vi "Set Control Translation.vi"(7 "Obj.":T2={"Type"=enum."Caption", "Translation ANSI"=[], "Translation Unicode"=[]}, 8 "error in (no error)":errorcluster, 9 "Default Lang":i32, 10 "Language":T1, 11 "Control in":refnum<vi>) -> (0 "error out":errorcluster, 3 "Unicode?":bool)   [LabVIEW 2019, in "Language Selection.lvlib"]
doc: "- - -\nCopyright (c) 2026, Merecs Engineering GmbH"
uses:
  Language Selection.lvlib
  TypeDefs/Cluster PropertyTranslation.ctl
  TypeDefs/Enum Property Type.ctl
  TypeDefs/Enum Language.ctl
  <vilib>/Utility/error.llb/Trim Whitespace.vi
  DVR Get Languages.vi
  <vilib>/addons/Tools/Unicode/_subVIs/Convert ASCII to UTF-16LE (1D).vi
  <vilib>/addons/Tools/Unicode/UI Unicode Tools.lvlib
  packages/error-generation/src/Error Generation/Error Generation.lvlib
panel:
  # "Connector Pane"
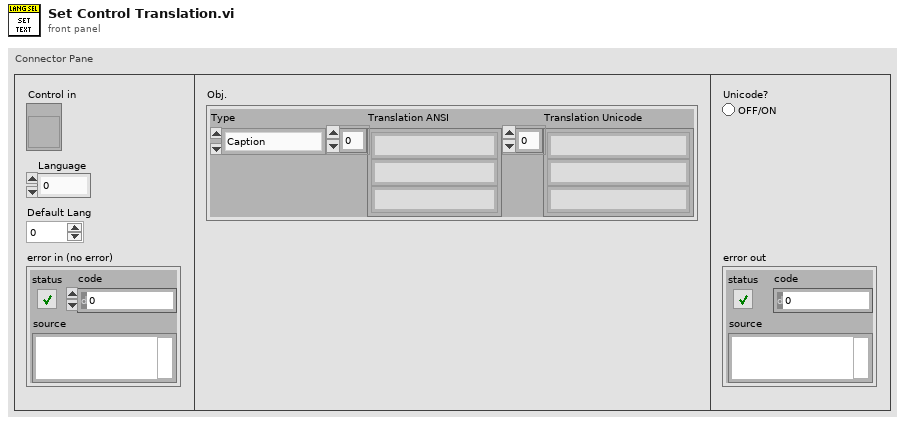
[diagram p1: front panel]
types:
  T1 = typedef "Language Selection.lvlib/Enum Language.ctl" = i32
  T2 = typedef "Language Selection.lvlib/Cluster PropertyTranslation.ctl" = cluster{"Type":T3, "Translation ANSI":string[], "Translation Unicode":string[]}
  T3 = typedef "Language Selection.lvlib/Enum Property Type.ctl" = enum16{"NA", "Caption", "String Value", "Boolean Text", "Ring Strings", "1D Array Elements", "2D Array Elements", "(MC)Listbox Header", "(MC)Listbox Items", "Tab Pages Names", "X & Y GraphChart", "Plot Names", "Table Headers", "Table Items", "TipStrip", "Combobox Strings", "Cursor Name", "Tree Col Headers"}
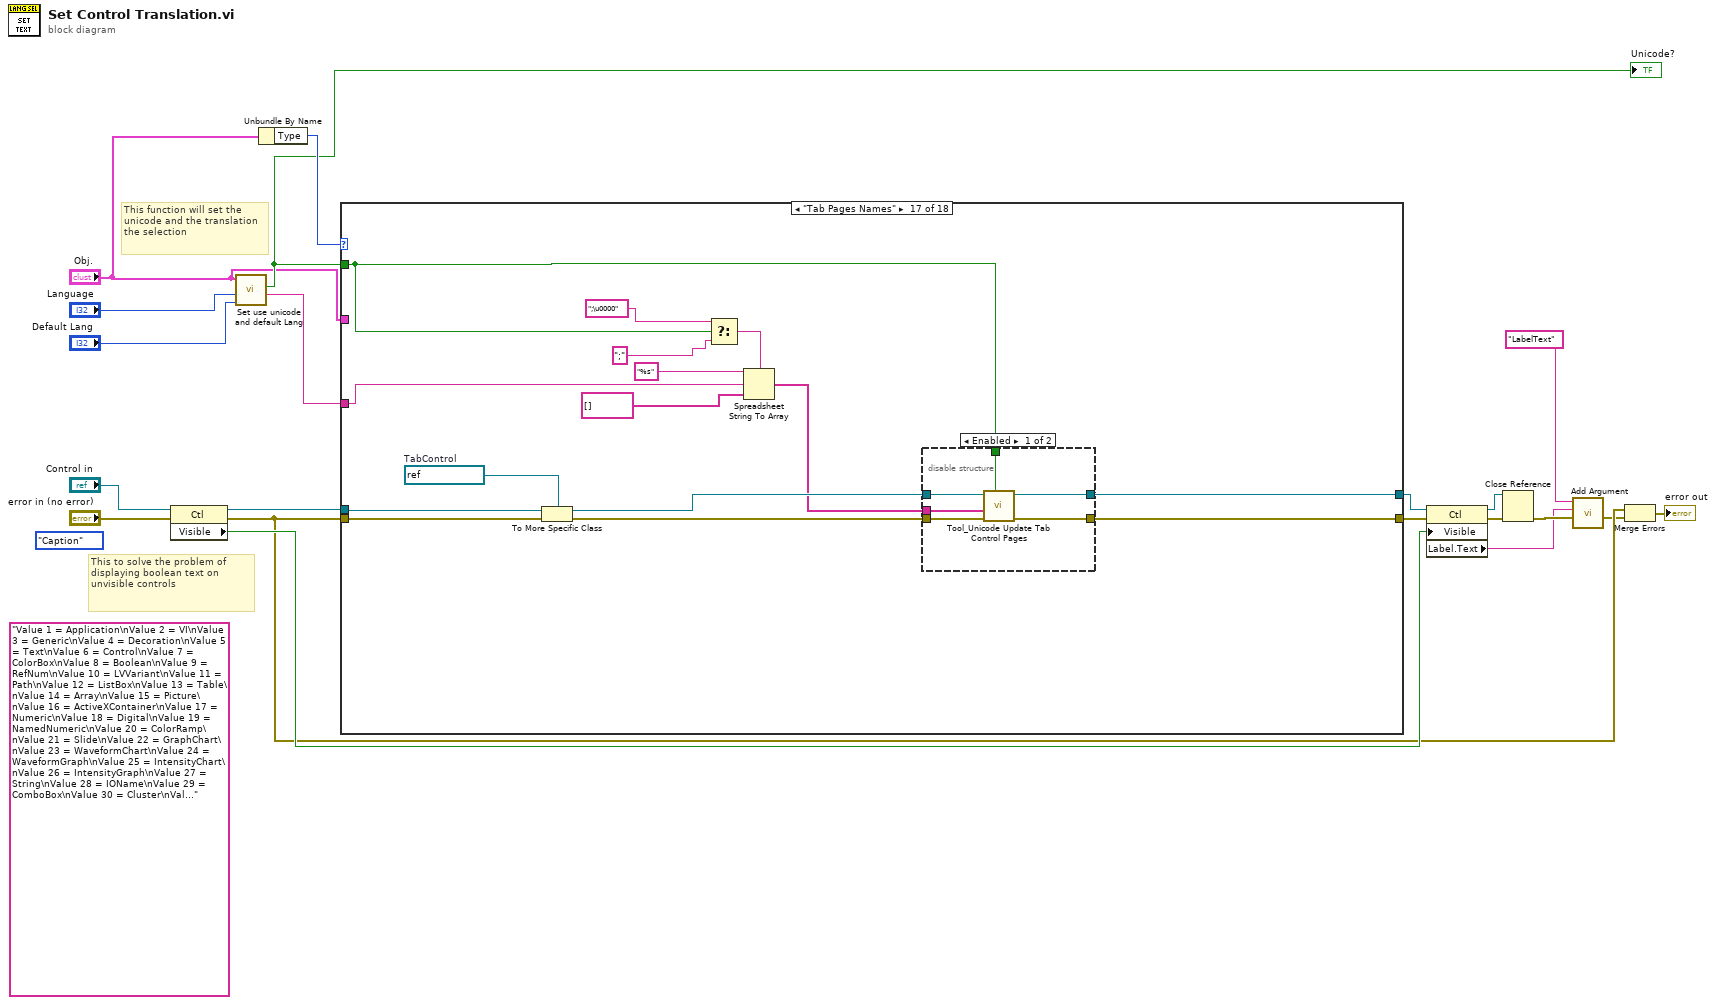
[diagram p0: block diagram]
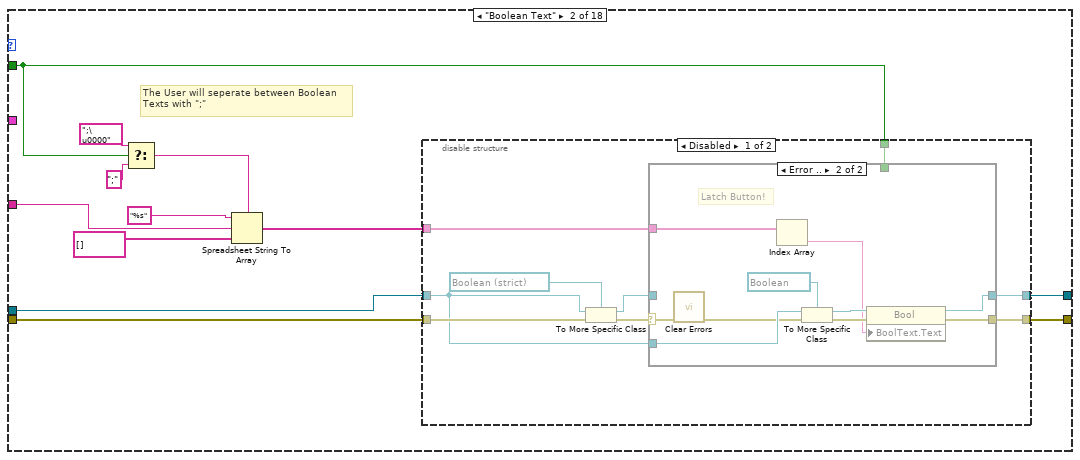
[diagram p3: hidden frame]
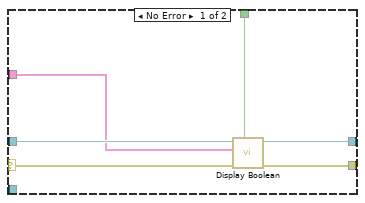
[diagram p4: hidden frame]
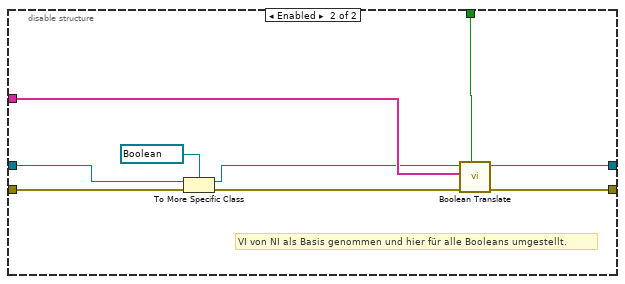
[diagram p5: hidden frame]
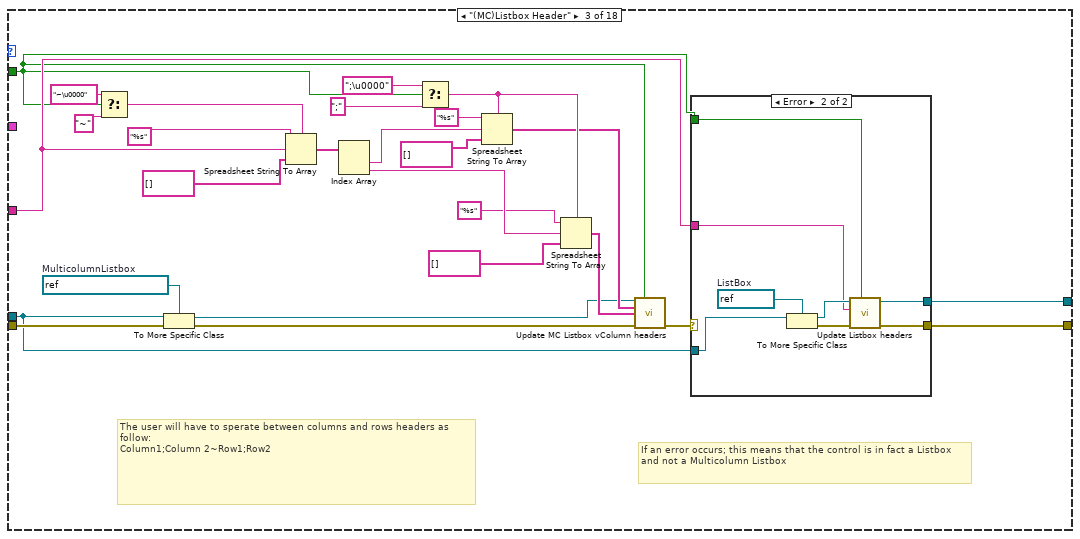
[diagram p6: hidden frame]
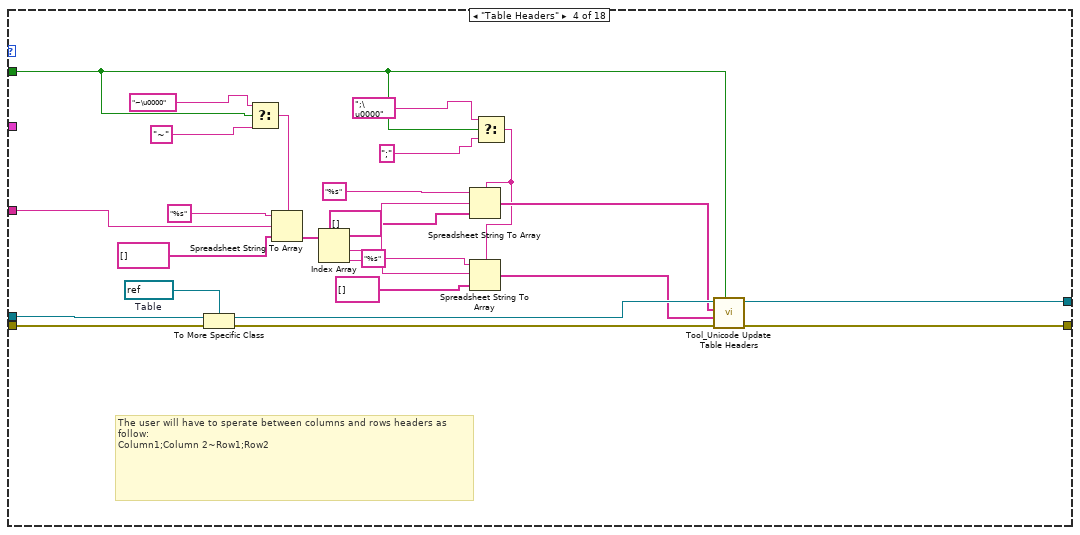
[diagram p8: hidden frame]
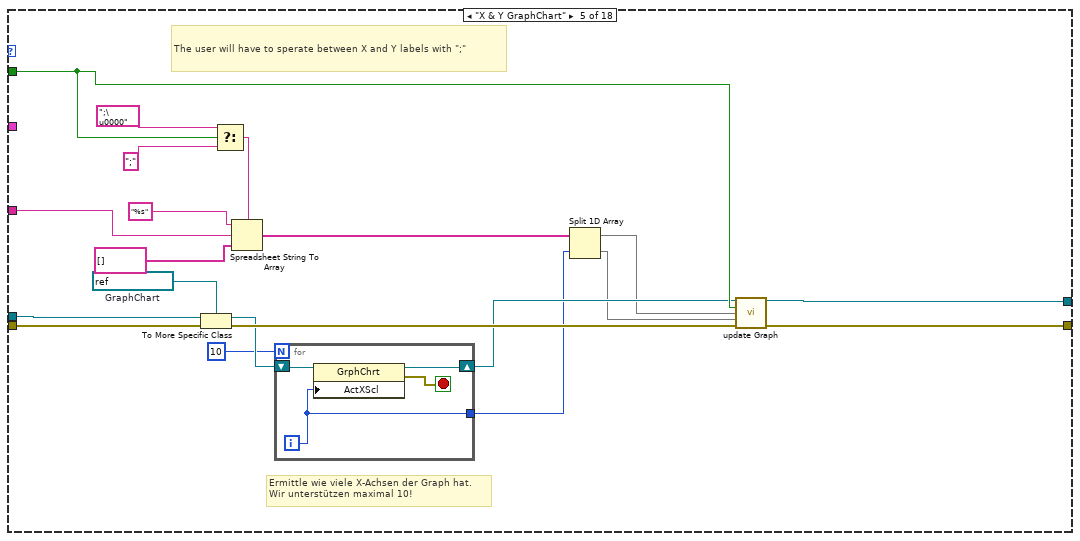
[diagram p9: hidden frame]
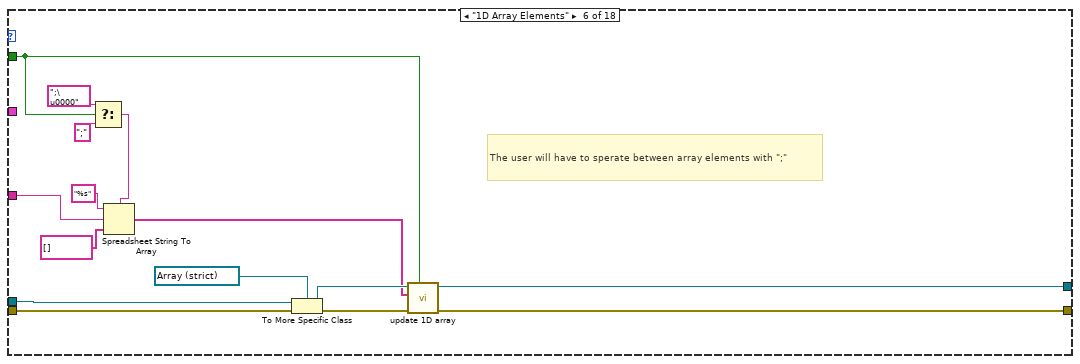
[diagram p10: hidden frame]
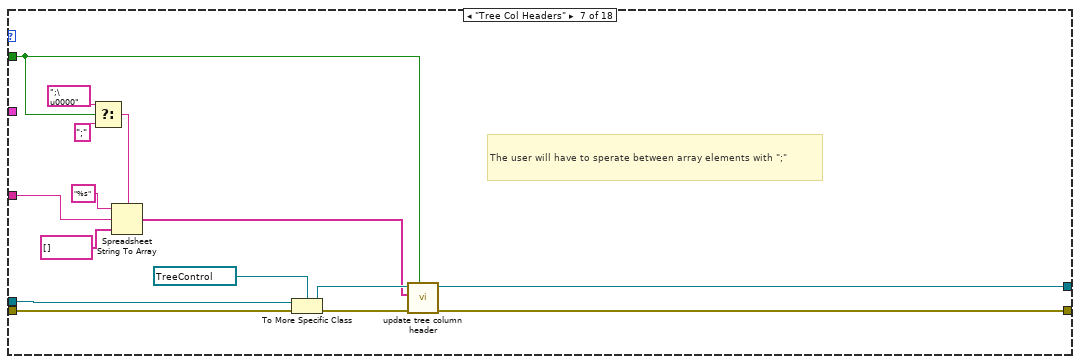
[diagram p11: hidden frame]
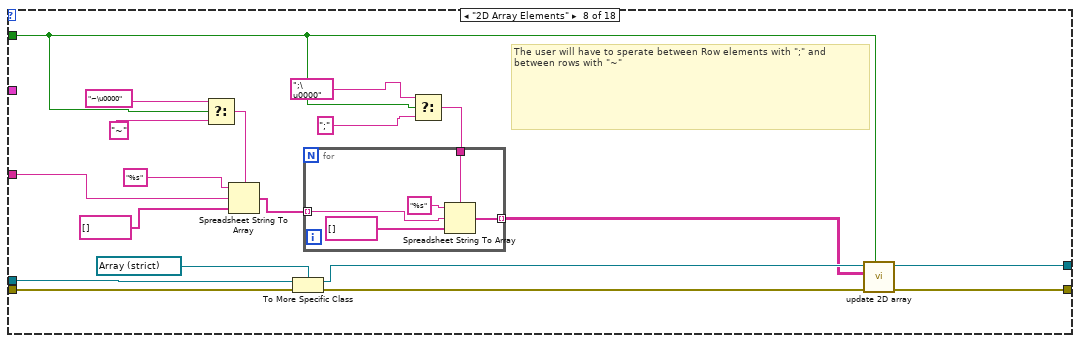
[diagram p12: hidden frame]
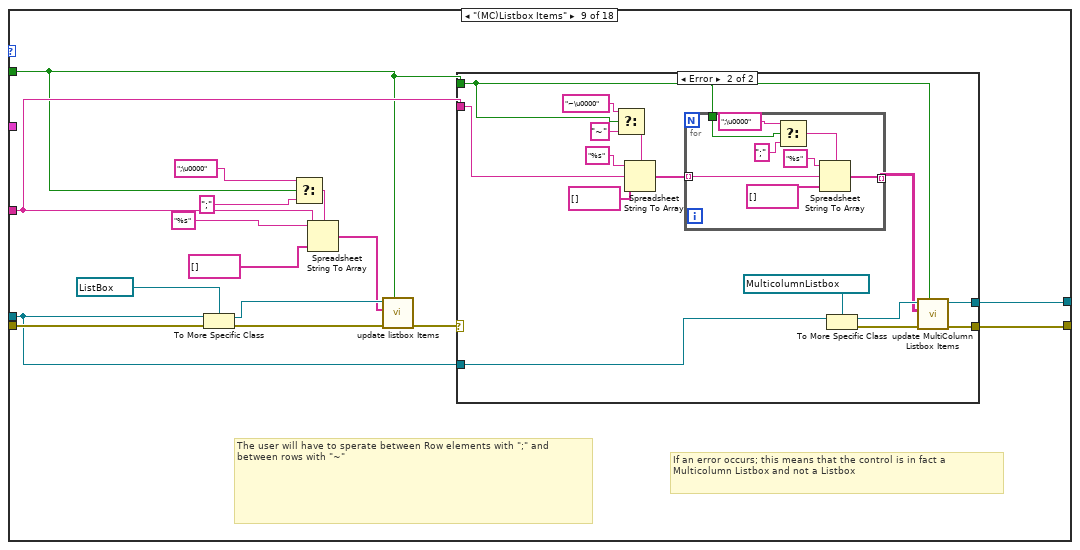
[diagram p13: hidden frame]
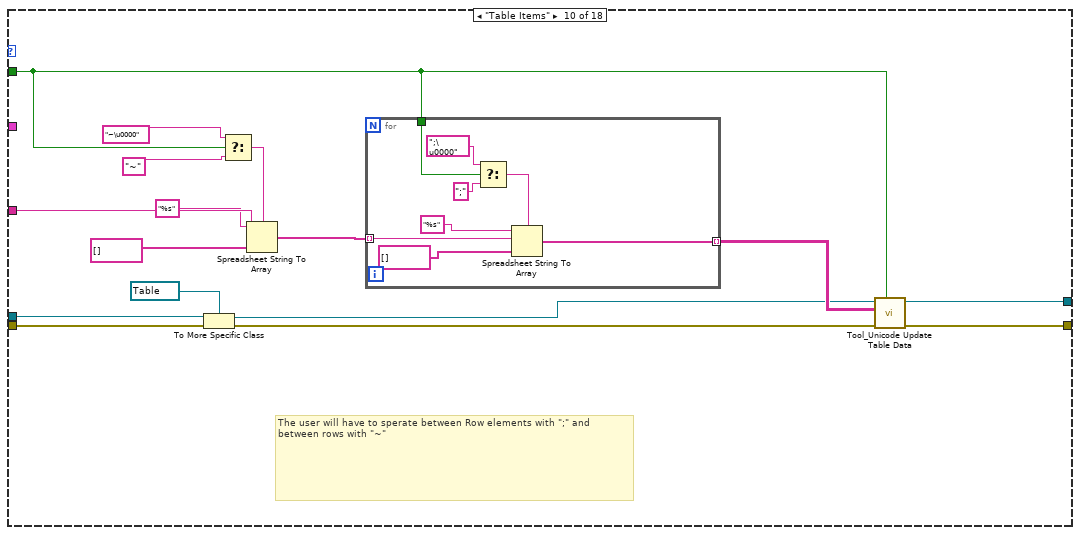
[diagram p15: hidden frame]
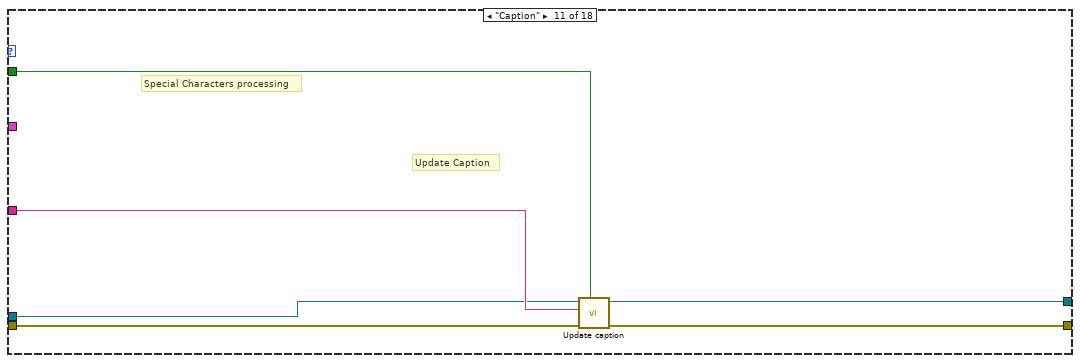
[diagram p16: hidden frame]
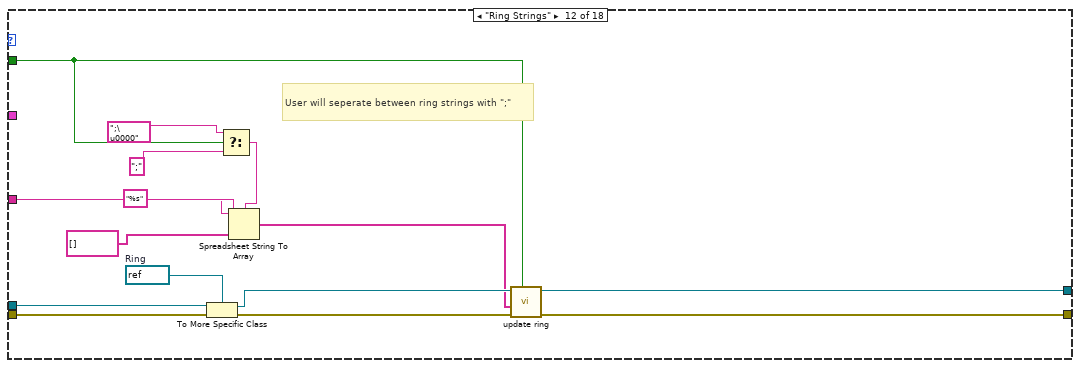
[diagram p17: hidden frame]
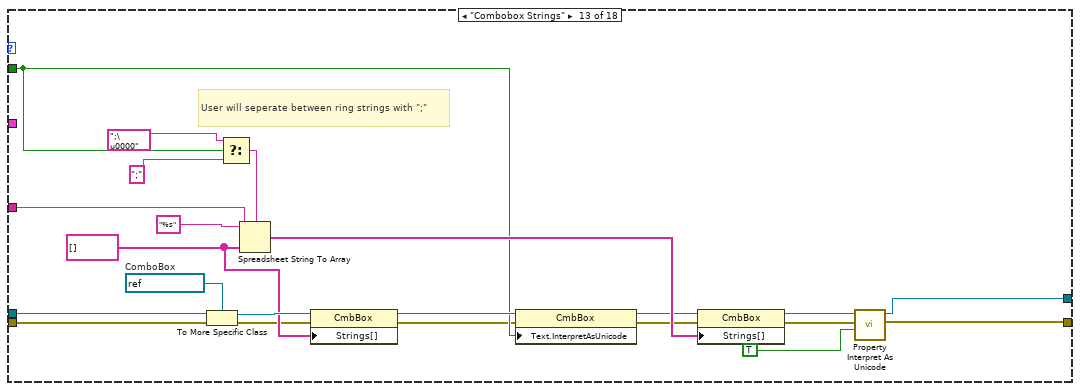
[diagram p18: hidden frame]
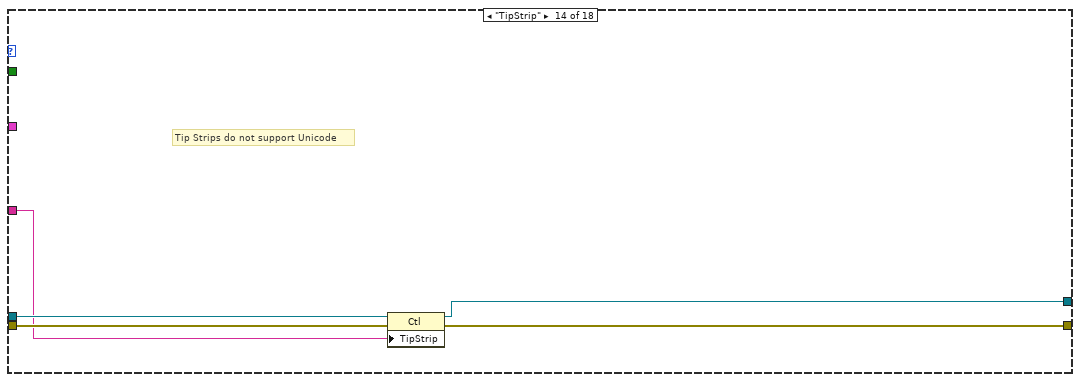
[diagram p19: hidden frame]
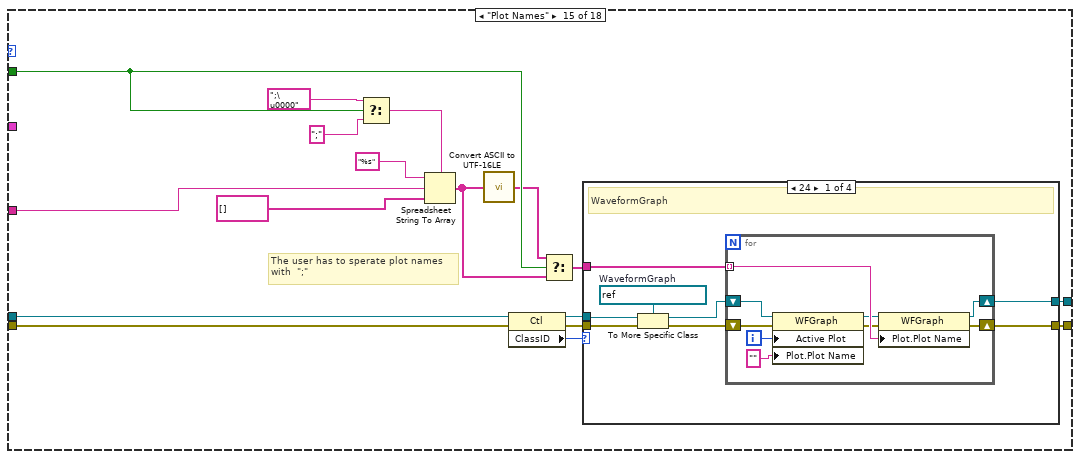
[diagram p20: hidden frame]
diagram:
  (unwired) "Value 1 = Application\nValue 2 = VI\nValue 3 = Generic\nValue 4 = Decoration\nValue 5 = Text\nValue 6 = Control\nValue 7 = ColorBox\nValue 8 = Boolean\nValue 9 = RefNum\nValue 10 = LVVariant\nValue 11 = Path\nValue 12 = ListBox\nValue 13 = Table\nValue 14 = Array\nValue 15 = Picture\nValue 16 = ActiveXContainer\nValue 17 = Numeric\nValue 18 = Digital\nValue 19 = NamedNumeric\nValue 20 = ColorRamp\nValue 21 = Slide\nValue 22 = GraphChart\nValue 23 = WaveformChart\nValue 24 = WaveformGraph\nValue 25 = IntensityChart\nValue 26 = IntensityGraph\nValue 27 = String\nValue 28 = IOName\nValue 29 = ComboBox\nValue 30 = Cluster\nValue 31 = Panel\nValue 32 = Knob\nValue 33 = NumericWithScale\nValue 34 = Ring\nValue 35 = Enum\nValue 36 = GObject\nValue 37 = Plot\nValue 38 = Cursor\nValue 39 = NumericText\nValue 40 = Scale\nValue 41 = ColorScale\nValue 42 = GraphScale\nValue 43 = ColorGraphScale\nValue 44 = TypedRefNum\nValue 45 = Generic\nValue 46 = MulticolumnListbox\nValue 47 = WaveformData\nValue 48 = DSCTag\nValue 49 = DAQChannelName\nValue 50 = VISAResourceName\nValue 51 = IVILogicalName\nValue 52 = SlideScale\nValue 53 = PageSelector\nValue 54 = Page\nValue 55 = TabControl\nValue 56 = ConnectorPane\nValue 57 = DAQmxName\nValue 58 = VIRefNum\nValue 59 = LVObjectRefNum\nValue 60 = AbsTime\nValue 61 = DigitalTable\nValue 62 = SubsystemVI\nValue 63 = Generic\nValue 64 = Generic\nValue 65 = SubPanel\nValue 66 = TreeControl\nValue 67 = GenClassTagRef\nValue 68 = GenClassRef\nValue 69 = RotaryColorScale\nValue 70 = PlugInControl\nValue 71 = PlugInDDODummyContainer\nValue 72 = RadioButtonsControl\nValue 73 = Project\nValue 74 = ProjectItem\nValue 75 = Pane\nValue 76 = Splitter\nValue 77 = BuildSpecification\nValue 78 = Pixmap\nValue 79 = FacadeVI\nValue 80 = Library\nValue 81 = Variable\nValue 82 = TagSet\nValue 83 = XYGraph\nValue 84 = SceneWindow\nValue 85 = LVClassLibrary\nValue 86 = Generic\nValue 87 = MethodVI\nValue 88 = XControlLibrary\nValue 89 = XNodeLibrary\nValue 90 = Scrollbar\nValue 91 = LVTarget\nValue 92 = MixedSignalGraph\nValue 93 = Provider\nValue 94 = CopyOperation\nValue 95 = TargetItem\nValue 96 = ProjectItemType\nValue 97 = CopyItem\nValue 98 = CopyConflict\nValue 99 = CopyExpert\nValue 100 = SceneGraphDisplay\nValue 101 = PolymorphicVI\nValue 102 = LabVIEWClassControl\nValue 103 = XInterfaceLibrary\nValue 104 = SceneNode\nValue 105 = SceneObject\nValue 106 = SceneLight\nValue 107 = Generic\nValue 108 = Generic\nValue 109 = Generic\nValue 110 = SceneClipPlane\nValue 111 = SceneTexture\nValue 112 = SceneGeometry\nValue 113 = SceneBox\nValue 114 = SceneCone\nValue 115 = SceneCylinder\nValue 116 = SceneHeightField\nValue 117 = SceneSphere\nValue 118 = SceneMesh\nValue 119 = XPropertyFolder\nValue 120 = PropertyFolder\nValue 121 = DigitalGraph\nValue 122 = GenClassTagFlatRef\nValue 123 = Scene\nValue 124 = Generic\nValue 125 = LibraryData\nValue 126 = StatechartLibrary\nValue 127 = MixedCheckbox\nValue 128 = SceneDrawable\nValue 129 = SceneText\nValue 130 = MultiSegmentPipe\nValue 131 = Bus\nValue 132 = StubDDO\nValue 133 = ProjectFilesViewItem\nValue 134 = LVClassPropDefFolder\nValue 135 = DataValRefNum"
  (unwired) Enum_Property_Type."Caption" ("Type")
  # "This to solve the problem of displaying boolean text on unvisible controls"
  # "This function will set the unicode and the translation the selection"
  n1 = property class="Ctl"(reference="Control in", error in="error in (no error)") -> (reference out=w13:refnum<vi>, error out=w7:errorcluster, "Visible"=w15:bool)
  n2 = call "Set use unicode and default Lang.vi"("Default Language"="Default Lang", "Startup Language"="Language", "Obj."="Obj.") -> ("Translation out"=w12:string, "Unicode?"=w11:bool)  [unwired: 7 in]
  "Unicode?" <- w11
  n3 = Unbundle By Name("Obj.") -> ("Type"=w20:T3)
  n4 = case shown="\"Tab Pages Names\"" w20 {
    tunnel: w12 -> [_ w33 w89 w127 w145 w168 w183 w203 w217 w265 w277 w288 w313 w318 w323 w411 w423 w447]
    tunnel: w13 -> [w21 w23 w79 w126 w150 w166 w181 w200 w218 w266 w275 w291 w315 w320 w336 w414 w429 w457]
    tunnel: w7 -> [w22 w24 w88 w125 w149 w165 w180 w199 w220 w258 w276 w293 w316 w319 w333 w416 w431 w458]
    tunnel: [w21 w26 w91 w121 w143 w162 w177 w195 w216 w257 w280 w295 w296 w322 w324 w409 w421 w453] -> w18
    tunnel: [w22 w25 w90 w128 w142 w161 w176 w194 w215 w255 w279 w294 w297 w321 w331 w408 w420 w454] -> w19
    tunnel: w11 -> [_ w27 w73 w107 w138 w156 w171 w186 w210 w251 w278 w282 w305 _ w339 w410 w417 w445]
    tunnel: "Obj." -> [_ _ _ _ _ _ _ _ _ _ _ _ _ _ _ _ _ _]
    frame "NA" {
    }
    frame "Boolean Text" {
      # "The User will seperate between Boolean\nTexts with \";\""
      n5 = Select(t=";\u0000" ("delimiter (Tab)"), s=w27, f=";" ("delimiter (Tab)")) -> (s? t:f=w31:string)
      n6 = Spreadsheet String To Array(delimiter (Tab)=w31, format string="%s", spreadsheet string=w33, array type (2D Dbl)=string[] [] ("Strings []")) -> (array=w28:string[])
      n7 = disable-structure shown="Disabled" {
        disable-tunnel: w23 -> [w35 w62]
        disable-tunnel: w28 -> [w43 w68]
        disable-tunnel: w27 -> [w42 w67]
        disable-tunnel: [w41 w66] -> w26
        disable-tunnel: [w40 w65] -> w25
        disable-tunnel: w24 -> [w39 w61]
        frame Disabled {
          n8 = To More Specific Class(target class=refnum<vi> refnum ("Boolean Reference"), reference=w35, error in=w39) -> (specific class reference=w36:refnum<vi>, error out=w38:errorcluster)
          n9 = case shown="Error .." w38 {
            selector: w38 -> [w44 w53]
            tunnel: w36 -> [w49 _]
            tunnel: w43 -> [w48 w51]
            tunnel: w42 -> [w47 _]
            tunnel: [w46 w54] -> w41
            tunnel: [w45 w55] -> w40
            tunnel: w35 -> [_ w56]
            frame No Error {
              n10 = call <vilib>:"Display Boolean.vi"("Interpret as Unicode (T)"=w47, "error in"=w44, "Boolean Texts [4]"=w48, "Boolean Reference"=w49) -> ("error out"=w45:errorcluster, "Boolean Reference"=w46:refnum<vi>)  [unwired: 4 in]
            }
            frame Error {
              # "Latch Button!"
              n11 = call <vilib>:"Clear Errors.vi"("error in (no error)"=w53) -> ("error out"=w52:errorcluster)  [unwired: 5 in, 1 out]
              n12 = Index Array(array=w51) -> (element=w50:string)  [unwired: 1 in]
              n13 = To More Specific Class(target class=refnum<vi> refnum ("Boolean Reference"), reference=w56, error in=w52) -> (specific class reference=w58:refnum<vi>, error out=w59:errorcluster)
              n14 = property class="Bool"(reference=w58, error in=w59, "BoolText.Text"=w50) -> (reference out=w54:refnum<vi>, error out=w55:errorcluster)
            }
          }
        }
        frame Enabled {
          # "VI von NI als Basis genommen und hier für alle Booleans umgestellt."
          n15 = To More Specific Class(target class=refnum<vi> refnum ("Boolean Reference"), reference=w62, error in=w61) -> (specific class reference=w63:refnum<vi>, error out=w60:errorcluster)
          n16 = call "Boolean Translate.vi"("Interpret as Unicode (T)"=w67, "error in"=w60, "Boolean Texts [4]"=w68, "Boolean Reference"=w63) -> ("error out"=w65:errorcluster, "Boolean Reference"=w66:refnum<vi>)  [unwired: 4 in]
        }
      }
    }
    frame "(MC)Listbox Header" {
      w94 = refnum<vi> refnum  # MulticolumnListbox
      # "If an error occurs; this means that the control is in fact a Listbox and not a Multicolumn Listbox"
      # "The user will have to sperate between columns and rows headers as follow:\nColumn1;Column 2~Row1;Row2"
      n17 = Select(t="~\u0000" ("delimiter (Tab)"), s=w73, f="~" ("delimiter (Tab)")) -> (s? t:f=w76:string)
      n18 = To More Specific Class(target class=w94, reference=w79, error in=w88) -> (specific class reference=w69:refnum<vi>, error out=w95:errorcluster)
      n19 = Spreadsheet String To Array(delimiter (Tab)=w76, format string="%s", spreadsheet string=w89, array type (2D Dbl)=string[] [] ("Strings []")) -> (array=w87:string[])
      n20 = Index Array(array=w87) -> (element #1=w86:string, element #2=w85:string)  [unwired: 2 in]
      n21 = Select(t=";\u0000" ("delimiter (Tab)"), s=w73, f=";" ("delimiter (Tab)")) -> (s? t:f=w72:string)
      n22 = Spreadsheet String To Array(delimiter (Tab)=w72, format string="%s", spreadsheet string=w86, array type (2D Dbl)=string[] [] ("Strings []")) -> (array=w71:string[])
      n23 = Spreadsheet String To Array(delimiter (Tab)=w72, format string="%s", spreadsheet string=w85, array type (2D Dbl)=string[] [] ("Strings []")) -> (array=w70:string[])
      n24 = call "Update MC Listbox vColumn headers.vi"("Multicolumn Listbox Ref"=w69, "Interpret as Unicode (T)"=w73, "Column Headers[]"=w71, "Row Headers[]"=w70, "Error in"=w95) -> ("error out"=w92:errorcluster)  [unwired: 9 in, 1 out]
      n25 = case shown="Error" w92 {
        selector: w92 -> [w97 _]
        tunnel: [w96 w103] -> w91
        tunnel: [w97 w101] -> w90
        tunnel: w89 -> [_ w98]
        tunnel: w73 -> [_ w100]
        tunnel: w79 -> [w96 w99]
        frame No Error {
        }
        frame Error {
          w105 = refnum<vi> refnum  # ListBox
          n26 = To More Specific Class(target class=w105, reference=w99) -> (specific class reference=w102:refnum<vi>, error out=w104:errorcluster)  [unwired: 1 in]
          n27 = call "Update Listbox headers.vi"("Interpret as Unicode (T)"=w100, "error in (no error)"=w104, "Column Header"=w98, "Listbox Ref"=w102) -> ("error out"=w101:errorcluster, "Listbox Ref"=w103:refnum<vi>)  [unwired: 6 in]
        }
      }
    }
    frame "Table Headers" {
      w130 = refnum<vi> refnum  # Table
      # "The user will have to sperate between columns and rows headers as follow:\nColumn1;Column 2~Row1;Row2"
      n28 = To More Specific Class(target class=w130, reference=w126, error in=w125) -> (specific class reference=w115:refnum<vi>, error out=w131:errorcluster)
      n29 = Select(t="~\u0000" ("delimiter (Tab)"), s=w107, f="~" ("delimiter (Tab)")) -> (s? t:f=w111:string)
      n30 = Spreadsheet String To Array(delimiter (Tab)=w111, format string="%s", spreadsheet string=w127, array type (2D Dbl)=string[] [] ("Strings []")) -> (array=w124:string[])
      n31 = Index Array(array=w124) -> (element #1=w123:string, element #2=w122:string)  [unwired: 2 in]
      n32 = Select(t=";\u0000" ("delimiter (Tab)"), s=w107, f=";" ("delimiter (Tab)")) -> (s? t:f=w106:string)
      n33 = Spreadsheet String To Array(delimiter (Tab)=w106, format string="%s", spreadsheet string=w123, array type (2D Dbl)=string[] [] ("Strings []")) -> (array=w114:string[])
      n34 = Spreadsheet String To Array(delimiter (Tab)=w106, format string="%s", spreadsheet string=w122, array type (2D Dbl)=string[] [] ("Strings []")) -> (array=w113:string[])
      n35 = call "Tool_Unicode Update Table Headers.vi"("Interpret as Unicode (T)"=w107, "error in (no error)"=w131, "Row Headers[]"=w113, "Column Headers[]"=w114, "Table Ref"=w115) -> ("error out"=w128:errorcluster, "Table Ref"=w121:refnum<vi>)  [unwired: 5 in]
    }
    frame "X & Y GraphChart" {
      w151 = refnum<vi> refnum  # GraphChart
      # "Ermittle wie viele X-Achsen der Graph hat.\nWir unterstützen maximal 10!"
      # "The user will have to sperate between X and Y labels with \";\""
      n36 = To More Specific Class(target class=w151, reference=w150, error in=w149) -> (specific class reference=w137:refnum<vi>, error out=w148:errorcluster)
      n37 = Select(t=";\u0000" ("delimiter (Tab)"), s=w138, f=";" ("delimiter (Tab)")) -> (s? t:f=w139:string)
      n38 = Spreadsheet String To Array(delimiter (Tab)=w139, format string="%s", spreadsheet string=w145, array type (2D Dbl)=string[] [] ("Strings []")) -> (array=w144:string[])
      n39 = for {
        N: 10 -> [_]
        shift-right: [w154] -> w136
        shift-left: w137 -> [w155]
        tunnel: [w152] -> w134
        i -> [w152]
        stop <- w153 stop-if-true
        n40 = property class="GrphChrt"(reference=w155, "ActXScl"=w152) -> (reference out=w154:refnum<vi>, error out=w153:errorcluster)  [unwired: 1 in]
      }
      n41 = Split 1D Array(array=w144, index=w134) -> (first subarray=w133:string[], second subarray=w132:string[])
      n42 = call "update Graph.vi"("GrphChrt Ref In"=w136, "Interpret as Unicode (T)"=w138, "X Axis Label"=w133, "Y Axis Label"=w132, "error in (no error)"=w148) -> ("GrphChrt Ref Out"=w143:refnum<vi>, "error out"=w142:errorcluster)  [unwired: 9 in]
    }
    frame "1D Array Elements" {
      # "The user will have to sperate between array elements with \";\""
      n43 = Select(t=";\u0000" ("delimiter (Tab)"), s=w156, f=";" ("delimiter (Tab)")) -> (s? t:f=w157:string)
      n44 = Spreadsheet String To Array(delimiter (Tab)=w157, format string="%s", spreadsheet string=w168, array type (2D Dbl)=string[] []) -> (array=w160:string[])
      n45 = To More Specific Class(target class=refnum<vi> refnum ("Arr Refnum"), reference=w166, error in=w165) -> (specific class reference=w164:refnum<vi>, error out=w163:errorcluster)
      n46 = call "update 1D array.vi"("Interpret as Unicode (T)"=w156, "error in (no error)"=w163, "Value"=w160, "String Array (1D) Ref In"=w164) -> ("error out"=w161:errorcluster, "String Array (1D) Ref Out"=w162:refnum<vi>)  [unwired: 6 in]
    }
    frame "Tree Col Headers" {
      # "The user will have to sperate between array elements with \";\""
      n47 = Select(t=";\u0000" ("delimiter (Tab)"), s=w171, f=";" ("delimiter (Tab)")) -> (s? t:f=w172:string)
      n48 = Spreadsheet String To Array(delimiter (Tab)=w172, format string="%s", spreadsheet string=w183, array type (2D Dbl)=string[] []) -> (array=w175:string[])
      n49 = To More Specific Class(target class=refnum<vi> refnum ("Tree Refnum"), reference=w181, error in=w180) -> (specific class reference=w179:refnum<vi>, error out=w178:errorcluster)
      n50 = call "update tree column header.vi"("Interpret as Unicode (T)"=w171, "error in (no error)"=w178, "Column Header"=w175, "Tree Refnum in"=w179) -> ("error out"=w176:errorcluster, "Tree Refnum out"=w177:refnum<vi>)  [unwired: 6 in]
    }
    frame "2D Array Elements" {
      # "The user will have to sperate between Row elements with \";\" and between rows with \"~\""
      n51 = Select(t="~\u0000" ("delimiter (Tab)"), s=w186, f="~" ("delimiter (Tab)")) -> (s? t:f=w190:string)
      n52 = Spreadsheet String To Array(delimiter (Tab)=w190, format string="%s", spreadsheet string=w203, array type (2D Dbl)=string[] []) -> (array=w201:string[])
      n53 = To More Specific Class(target class=refnum<vi> refnum ("Control in 2"), reference=w200, error in=w199) -> (specific class reference=w197:refnum<vi>, error out=w196:errorcluster)
      n54 = Select(t=";\u0000" ("delimiter (Tab)"), s=w186, f=";" ("delimiter (Tab)")) -> (s? t:f=w187:string)
      n55 = for {
        tunnel: w201 -> [w207] mode=indexing
        tunnel: [w206] -> w193 mode=indexing
        tunnel: w187 -> [w205]
        n56 = Spreadsheet String To Array(delimiter (Tab)=w205, format string="%s", spreadsheet string=w207, array type (2D Dbl)=string[] []) -> (array=w206:string[])
      }
      n57 = call "update 2D array.vi"("Interpret as Unicode (T)"=w186, "error in (no error)"=w196, "Value"=w193, "String Array (2D) Ref"=w197) -> ("error out"=w194:errorcluster, "String Array (2D) Ref"=w195:refnum<vi>)  [unwired: 6 in]
    }
    frame "(MC)Listbox Items" {
      # "The user will have to sperate between Row elements with \";\" and between rows with \"~\""
      # "If an error occurs; this means that the control is in fact a Multicolumn Listbox and not a Listbox"
      n58 = To More Specific Class(target class=refnum<vi> refnum ("Listbox Ref"), reference=w218, error in=w220) -> (specific class reference=w222:refnum<vi>, error out=w221:errorcluster)
      n59 = Select(t=";\u0000" ("delimiter (Tab)"), s=w210, f=";" ("delimiter (Tab)")) -> (s? t:f=w211:string)
      n60 = Spreadsheet String To Array(delimiter (Tab)=w211, format string="%s", spreadsheet string=w217, array type (2D Dbl)=string[] []) -> (array=w214:string[])
      n61 = call "update listbox Items.vi"("Unicode?"=w210, "error in (no error)"=w221, "Data[]"=w214, "Listbox Ref"=w222) -> ("error out"=w219:errorcluster)  [unwired: 6 in, 1 out]
      n62 = case shown="Error" w219 {
        selector: w219 -> [w226 _]
        tunnel: w218 -> [w227 w241]
        tunnel: w217 -> [_ w237]
        tunnel: w210 -> [_ w228]
        tunnel: [w227 w234] -> w216
        tunnel: [w226 w233] -> w215
        frame No Error {
        }
        frame Error {
          n63 = Select(t="~\u0000" ("delimiter (Tab)"), s=w228, f="~") -> (s? t:f=w229:string)
          n64 = Spreadsheet String To Array(delimiter (Tab)=w229, format string="%s", spreadsheet string=w237, array type (2D Dbl)=string[] []) -> (array=w236:string[])
          n65 = for {
            tunnel: w236 -> [w248] mode=indexing
            tunnel: [w247] -> w232 mode=indexing
            tunnel: w228 -> [w246]
            n66 = Select(t=";\u0000" ("delimiter (Tab)"), s=w246, f=";" ("delimiter (Tab)")) -> (s? t:f=w243:string)
            n67 = Spreadsheet String To Array(delimiter (Tab)=w243, format string="%s", spreadsheet string=w248, array type (2D Dbl)=string[] []) -> (array=w247:string[])
          }
          n68 = To More Specific Class(target class=refnum<vi> refnum ("Multicolumn Listbox Ref"), reference=w241) -> (specific class reference=w240:refnum<vi>, error out=w235:errorcluster)  [unwired: 1 in]
          n69 = call "update MultiColumn Listbox Items.vi"("Interpret as Unicode (T)"=w228, "error in (no error)"=w235, "Data[]"=w232, "Multicolumn Listbox Ref"=w240) -> ("error out"=w233:errorcluster, "Multicolumn Listbox Ref"=w234:refnum<vi>)  [unwired: 6 in]
        }
      }
    }
    frame "Table Items" {
      # "The user will have to sperate between Row elements with \";\" and between rows with \"~\""
      n70 = To More Specific Class(target class=refnum<vi> refnum ("Multicolumn Listbox Ref"), reference=w266, error in=w258) -> (specific class reference=w259:refnum<vi>, error out=w256:errorcluster)
      n71 = Select(t="~\u0000" ("delimiter (Tab)"), s=w251, f="~" ("delimiter (Tab)")) -> (s? t:f=w252:string)
      n72 = Spreadsheet String To Array(delimiter (Tab)=w252, format string="%s", spreadsheet string=w265, array type (2D Dbl)=string[] []) -> (array=w261:string[])
      n73 = for {
        tunnel: w261 -> [w272] mode=indexing
        tunnel: [w271] -> w260 mode=indexing
        tunnel: w251 -> [w270]
        n74 = Select(t=";\u0000" ("delimiter (Tab)"), s=w270, f=";" ("delimiter (Tab)")) -> (s? t:f=w267:string)
        n75 = Spreadsheet String To Array(delimiter (Tab)=w267, format string="%s", spreadsheet string=w272, array type (2D Dbl)=string[] []) -> (array=w271:string[])
      }
      n76 = call "Tool_Unicode Update Table Data.vi"("Interpret as Unicode (T)"=w251, "error in (no error)"=w256, "Data[]"=w260, "Table Ref"=w259) -> ("error out"=w255:errorcluster, "Table Ref"=w257:refnum<vi>)  [unwired: 4 in]
    }
    frame "Caption" {
      # "Special Characters processing"
      # "Update Caption"
      n77 = call "Update caption.vi"("Interpret as Unicode (T)"=w278, "error in (no error)"=w276, "Caption In"=w277, "Control Reference In"=w275) -> ("error out"=w279:errorcluster, "Control Reference Out"=w280:refnum<vi>)  [unwired: 6 in]
    }
    frame "Ring Strings" {
      w289 = refnum<vi> refnum  # Ring
      # "User will seperate between ring strings with \";\""
      n78 = To More Specific Class(target class=w289, reference=w291, error in=w293) -> (specific class reference=w290:refnum<vi>, error out=w292:errorcluster)
      n79 = Select(t=";\u0000" ("delimiter (Tab)"), s=w282, f=";" ("delimiter (Tab)")) -> (s? t:f=w281:string)
      n80 = Spreadsheet String To Array(delimiter (Tab)=w281, format string="%s", spreadsheet string=w288, array type (2D Dbl)=string[] [] ("Strings []")) -> (array=w285:string[])
      n81 = call "update ring.vi"("Interpret as Unicode (T)"=w282, "error in (no error)"=w292, "Ring Texts"=w285, "Ring Control Ref"=w290) -> ("error out"=w294:errorcluster, "Ring Control Ref"=w295:refnum<vi>)  [unwired: 6 in]
    }
    frame "Combobox Strings" {
      w304 = string[] [] ("Strings []")
      w314 = refnum<vi> refnum  # ComboBox
      # "User will seperate between ring strings with \";\""
      n82 = To More Specific Class(target class=w314, reference=w315, error in=w316) -> (specific class reference=w308:refnum<vi>, error out=w303:errorcluster)
      n83 = Select(t=";\u0000" ("delimiter (Tab)"), s=w305, f=";" ("delimiter (Tab)")) -> (s? t:f=w309:string)
      n84 = Spreadsheet String To Array(delimiter (Tab)=w309, format string="%s", spreadsheet string=w313, array type (2D Dbl)=w304) -> (array=w317:string[])
      n85 = property class="CmbBox"(reference=w308, error in=w303, "Strings[]"=w304) -> (reference out=w307:refnum<vi>, error out=w301:errorcluster)
      n86 = property class="CmbBox"(reference=w307, error in=w301, "Text.InterpretAsUnicode"=w305) -> (reference out=w306:refnum<vi>, error out=w302:errorcluster)
      n87 = property class="CmbBox"(reference=w306, error in=w302, "Strings[]"=w317) -> (reference out=w300:refnum<vi>, error out=w298:errorcluster)
      n88 = call <vilib>:"Property Interpret As Unicode.vi"("Interpret As Unicode (T)"=TRUE, "error in (no error)"=w298, "String Control Reference"=w300) -> ("error out"=w297:errorcluster, "String Control Reference"=w296:refnum<vi>)  [unwired: 5 in]
    }
    frame "TipStrip" {
      # "Tip Strips do not support Unicode"
      n89 = property class="Ctl"(reference=w320, error in=w319, "TipStrip"=w318) -> (reference out=w322:refnum<vi>, error out=w321:errorcluster)
    }
    frame "Plot Names" {
      # "The user has to sperate plot names \nwith  \";\""
      n90 = Select(t=";\u0000" ("delimiter (Tab)"), s=w339, f=";" ("delimiter (Tab)")) -> (s? t:f=w329:string)
      n91 = Spreadsheet String To Array(delimiter (Tab)=w329, format string="%s", spreadsheet string=w323, array type (2D Dbl)=string[] [] ("Strings []")) -> (array=w326:string[])
      n92 = call-poly <vilib>:"Convert ASCII to UTF-16LE.vi"("ASCII"=w326) -> ("Unicode"=w325:string[])  [unwired: 4 in]
      n93 = property class="Ctl"(reference=w336, error in=w333) -> (reference out=w334:refnum<vi>, error out=w332:errorcluster, "ClassID"=w335:u32)
      n94 = Select(t=w325, s=w339, f=w326) -> (s? t:f=w327:string[])
      n95 = case shown="24" w335 {
        tunnel: w334 -> [w347 w364 w381 w398]
        tunnel: w332 -> [w346 w363 w380 w392]
        tunnel: [w341 w360 w378 w394] -> w331
        tunnel: [w342 w359 w377 w393] -> w324
        tunnel: w327 -> [w340 w358 w374 w391]
        frame 24 {
          w345 = refnum<vi> refnum  # WaveformGraph
          # "WaveformGraph"
          n96 = To More Specific Class(target class=w345, reference=w347, error in=w346) -> (specific class reference=w343:refnum<vi>, error out=w344:errorcluster)
          n97 = for {
            shift-right: [w348] -> w342
            shift-left: w343 -> [w355]
            shift-right: [w349] -> w341
            shift-left: w344 -> [w354]
            tunnel: w340 -> [w356] mode=indexing
            i -> [w353]
            n98 = property class="WFGraph"(reference=w355, error in=w354, "Active Plot"=w353, "Plot.Plot Name"="") -> (reference out=w351:refnum<vi>, error out=w350:errorcluster)
            n99 = property class="WFGraph"(reference=w351, error in=w350, "Plot.Plot Name"=w356) -> (reference out=w348:refnum<vi>, error out=w349:errorcluster)
          }
        }
        frame 83 {
          w362 = refnum<vi> refnum  # XYGraph
          # "XY Graph"
          n100 = To More Specific Class(target class=w362, reference=w364, error in=w363) -> (specific class reference=w361:refnum<vi>, error out=w357:errorcluster)
          n101 = for {
            shift-right: [w365] -> w359
            shift-left: w361 -> [w372]
            shift-right: [w366] -> w360
            shift-left: w357 -> [w371]
            tunnel: w358 -> [w373] mode=indexing
            i -> [w370]
            n102 = property class="XYGraph"(reference=w372, error in=w371, "Active Plot"=w370, "Plot.Plot Name"="") -> (reference out=w368:refnum<vi>, error out=w367:errorcluster)
            n103 = property class="XYGraph"(reference=w368, error in=w367, "Plot.Plot Name"=w373) -> (reference out=w365:refnum<vi>, error out=w366:errorcluster)
          }
        }
        frame 121 {
          w379 = refnum<vi> refnum  # DigitalGraph
          # "DigitalGraph"
          n104 = To More Specific Class(target class=w379, reference=w381, error in=w380) -> (specific class reference=w376:refnum<vi>, error out=w375:errorcluster)
          n105 = for {
            shift-right: [w382] -> w377
            shift-left: w376 -> [w389]
            shift-right: [w383] -> w378
            shift-left: w375 -> [w388]
            tunnel: w374 -> [w390] mode=indexing
            i -> [w387]
            n106 = property class="DigitalGraph"(reference=w389, error in=w388, "Active Plot"=w387, "Plot.Plot Name"="") -> (reference out=w385:refnum<vi>, error out=w384:errorcluster)
            n107 = property class="DigitalGraph"(reference=w385, error in=w384, "Plot.Plot Name"=w390) -> (reference out=w382:refnum<vi>, error out=w383:errorcluster)
          }
        }
        frame 23, Default {
          w397 = refnum<vi> refnum  # WaveformChart
          # "WaveformChart"
          n108 = To More Specific Class(target class=w397, reference=w398, error in=w392) -> (specific class reference=w396:refnum<vi>, error out=w395:errorcluster)
          n109 = for {
            shift-right: [w400] -> w393
            shift-left: w396 -> [w407]
            shift-right: [w401] -> w394
            shift-left: w395 -> [w406]
            tunnel: w391 -> [w399] mode=indexing
            i -> [w405]
            n110 = property class="WFChart"(reference=w407, error in=w406, "Active Plot"=w405, "Plot.Plot Name"="") -> (reference out=w403:refnum<vi>, error out=w402:errorcluster)
            n111 = property class="WFChart"(reference=w403, error in=w402, "Plot.Plot Name"=w399) -> (reference out=w400:refnum<vi>, error out=w401:errorcluster)
          }
        }
      }
    }
    frame "String Value" {
      w413 = refnum<vi> refnum  # String
      n112 = To More Specific Class(target class=w413, reference=w414, error in=w416) -> (specific class reference=w412:refnum<vi>, error out=w415:errorcluster)
      n113 = call "Update String value.vi"("Interpret as Unicode (T)"=w410, "error in (no error)"=w415, "String Value"=w411, "String Control Reference In"=w412) -> ("error out"=w408:errorcluster, "String Control Reference Out"=w409:refnum<vi>)  [unwired: 6 in]
    }
    frame "Tab Pages Names" {
      w428 = refnum<vi> refnum  # TabControl
      n114 = To More Specific Class(target class=w428, reference=w429, error in=w431) -> (specific class reference=w419:refnum<vi>, error out=w430:errorcluster)
      n115 = Select(t=";\u0000" ("delimiter (Tab)"), s=w417, f=";" ("delimiter (Tab)")) -> (s? t:f=w425:string)
      n116 = Spreadsheet String To Array(delimiter (Tab)=w425, format string="%s", spreadsheet string=w423, array type (2D Dbl)=string[] [] ("Strings []")) -> (array=w418:string[])
      n117 = disable-structure shown="Enabled" {
        disable-tunnel: w430 -> [w437 w440]
        disable-tunnel: [w436 w438] -> w421
        disable-tunnel: [w435 w439] -> w420
        disable-tunnel: w419 -> [w434 w442]
        disable-tunnel: w418 -> [w433 w441]
        disable-tunnel: w417 -> [w432 w443]
        frame Enabled {
          n118 = call "Tool_Unicode Update Tab Control Pages.vi"("Interpret as Unicode (T)"=w432, "error in (no error)"=w437, "Page Captions"=w433, "Tab Control"=w434) -> ("error out"=w435:errorcluster, "Tab Control"=w436:refnum<vi>)  [unwired: 4 in]
        }
        frame Disabled {
          # "This VI from NI has is bugi!"
          n119 = call <vilib>:"Update Tab Control Pages.vi"("Interpret as Unicode (T)"=w443, "error in"=w440, "Page Captions"=w441, "Tab Control"=w442) -> ("error out"=w439:errorcluster, "Tab Control"=w438:refnum<vi>)  [unwired: 4 in]
        }
      }
    }
    frame "Cursor Name" {
      w456 = refnum<vi> refnum  # WaveformGraph
      n120 = Select(t=";\u0000" ("delimiter (Tab)"), s=w445, f=";" ("delimiter (Tab)")) -> (s? t:f=w450:string)
      n121 = To More Specific Class(target class=w456, reference=w457, error in=w458) -> (specific class reference=w455:refnum<vi>, error out=w444:errorcluster)
      n122 = Spreadsheet String To Array(delimiter (Tab)=w450, format string="%s", spreadsheet string=w447, array type (2D Dbl)=string[] [] ("Strings []")) -> (array=w446:string[])
      n123 = case shown="No Error" w444 {
        selector: w444 -> [w459 w478]
        tunnel: w455 -> [w464 w479]
        tunnel: [w463 w477] -> w454
        tunnel: [w462 w479] -> w453
        tunnel: w446 -> [w461 _]
        tunnel: w445 -> [w460 _]
        frame No Error {
          n124 = for {
            shift-right: [w469] -> w462
            shift-left: w464 -> [w472]
            shift-right: [w470] -> w463
            shift-left: w459 -> [w471]
            tunnel: w460 -> [w467]
            tunnel: w461 -> [w466] mode=indexing
            i -> [w468]
            n125 = case shown="True" w467 {
              tunnel: w466 -> [w473 w475]
              tunnel: [w473 w474] -> w465
              frame False {
              }
              frame True {
                w476 = "ÿþ"  # Unicode Header
                n126 = Concatenate Strings(w476, w475) -> (w474:string)
              }
            }
            n127 = property on="Property Node" class="WFGraph"(reference=w472, error in=w471, "Active Cursor"=w468, "Cursor.Cursor Name"=w465) -> (reference out=w469:refnum<vi>, error out=w470:errorcluster)
          }
        }
        frame Error {
          # "Not a graph.\nThe graph only has cursor."
          n128 = call <vilib>:"Clear Errors.vi"("error in (no error)"=w478) -> ("error out"=w477:errorcluster)  [unwired: 5 in, 1 out]
        }
      }
    }
  }
  n129 = property class="Ctl"(reference=w18, error in=w19, "Visible"=w15) -> (reference out=w16:refnum<vi>, error out=w17:errorcluster, "Label.Text"=w5:string)
  n130 = Close Reference(reference=w16, error in (no error)=w17) -> (error out=w10:errorcluster)
  n131 = call "Add Argument.vi"("error in (no error)"=w10, "argument data"=w5, "argument"="LabelText") -> ("error out"=w6:errorcluster)  [unwired: 8 in]
  n132 = Merge Errors(w7, w6) -> (→"error out":errorcluster)
